vi "Conpane Caller A.vi"() -> (0 "Marker Out":dbl)   [LabVIEW 2026]
doc: "Round-13 counter-probe: calls Conpane Probe A.vi, the variant with NO conIdx and therefore no connector-pane terminals. Whatever this does - refuse to compose, or compose a Call with nothing to wire - is the failure mode of a pane-less subVI."
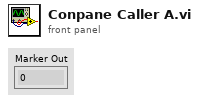
[diagram p1: front panel]
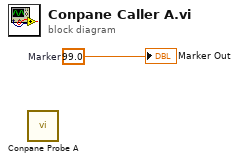
[diagram p0: block diagram]
diagram:
  w1 = 99.0  # Marker
  n1 = call "Conpane Probe A.vi"() -> ()  [unwired: 16 in]
  "Marker Out" <- w1
